vi "Func - LV runtime error handler.vi"(2 "InstanceRef":T1, 3 "error in":bool, 4 "Gen CE error?":bool, 5 "LabVIEW error code":i32) -> (0 "error out":bool)   [LabVIEW 2021]
doc: "This VI handles errors produced by LabVIEW VIs and functions.\n\nFor more information, see help for this VI.\n\n::: CalcExpress Toolkit :::\nCopyright (c) 2000-2026 Konstantin Shifershteyn. All rights reserved."
uses:
  cetypes.llb/CalcExpress Instance RefNum.ctl
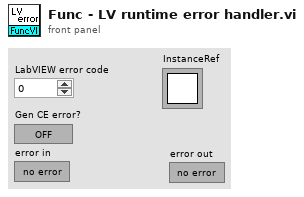
[diagram p1: front panel]
types:
  T1 = typedef "CalcExpress Instance RefNum.ctl" = refnum<k1>
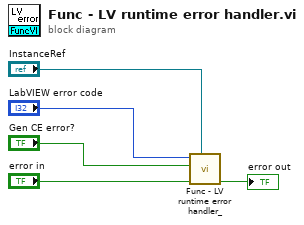
[diagram p0: block diagram]
diagram:
  n1 = call "Func - LV runtime error handler_.vi"("InstanceRef"="InstanceRef", "error in"="error in", "Gen CE error?"="Gen CE error?", "LabVIEW error code"="LabVIEW error code") -> ("error out"=→"error out":bool)  [unwired: 7 in]
